vi "Retest_Continue_NO.vi"(8 "error in":errorcluster, 9 "Enable":bool=TRUE, 10 "input string":string, 11 "Text.Text Colors:BG Color":u32(colorbox)=16448250) -> (0 "error out":errorcluster, 1 "Boolean":bool, 2 "Continue 2":bool)   [LabVIEW 2021]
panel:
  in  "Continue":bool caption="Enter to continue"
  in  "Cancel":bool caption="ESC to No"
  in  "OK Button":bool caption="F3 to Retest"
  out "String":string
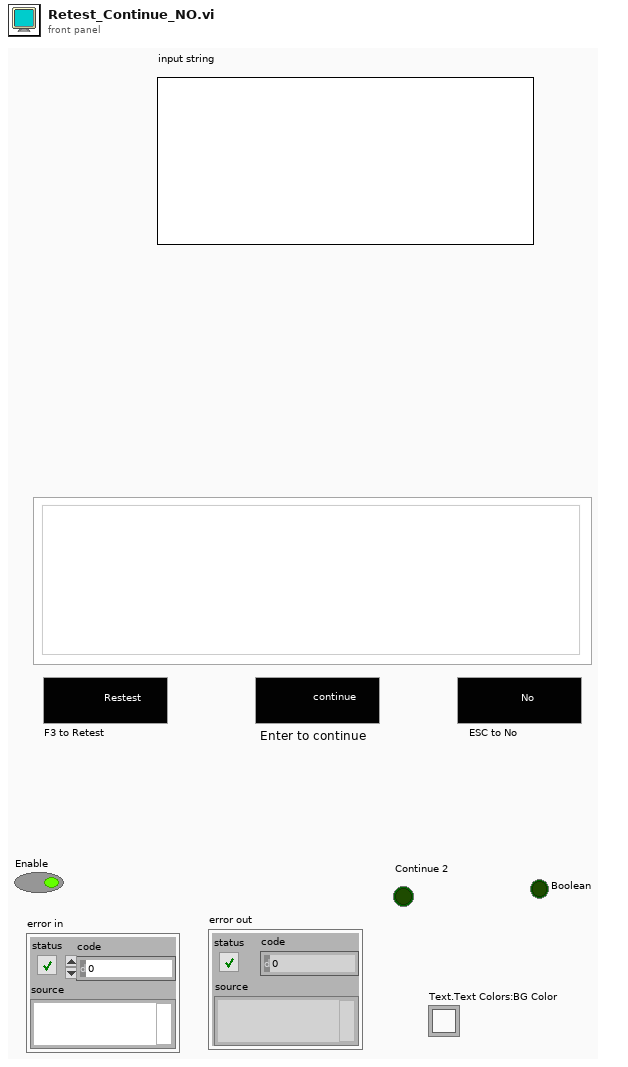
[diagram p1: front panel]
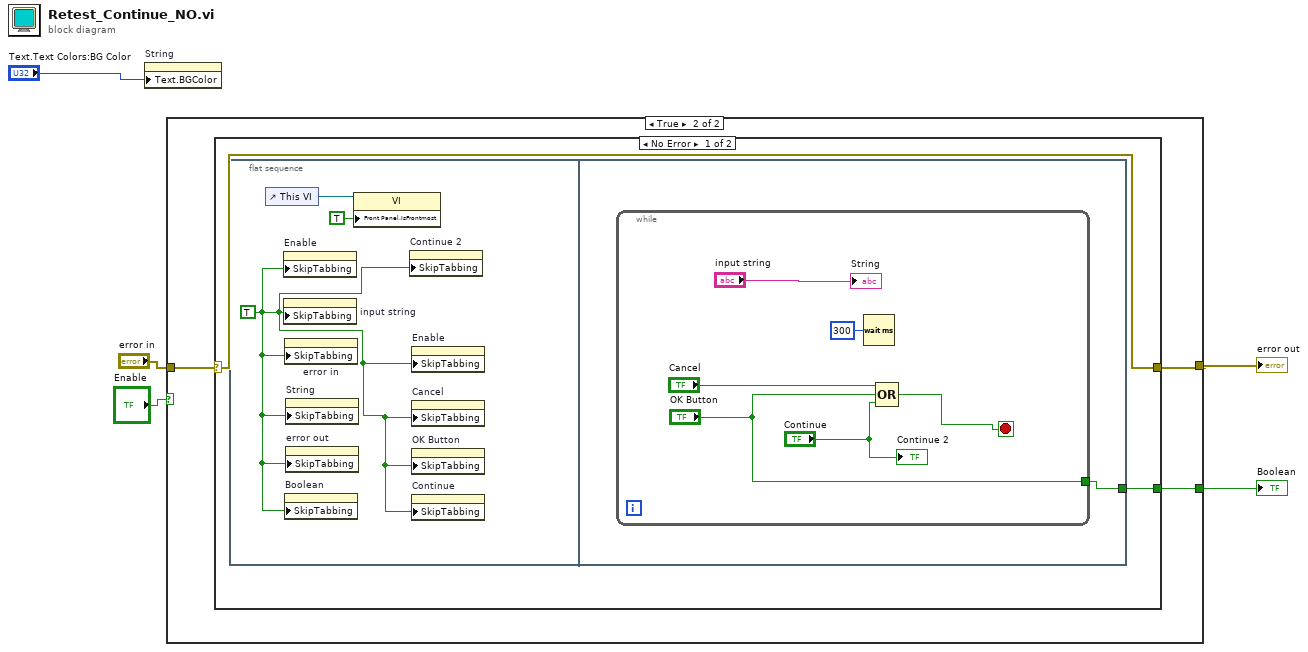
[diagram p0: block diagram]
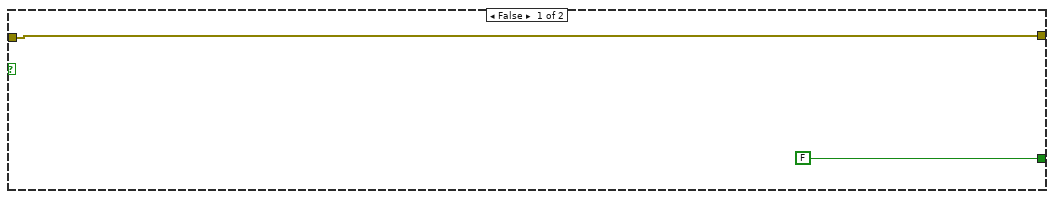
[diagram p2: hidden frame]
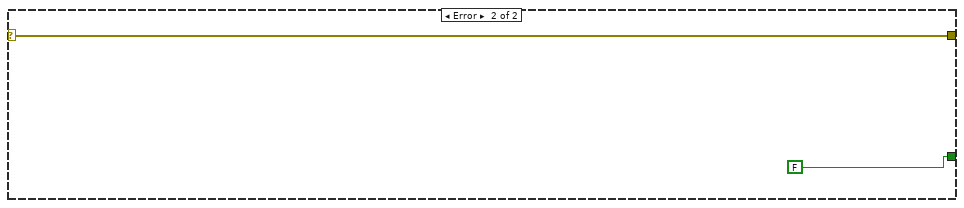
[diagram p3: hidden frame]
diagram:
  n1 = property on="String" class="Str"("Text.BGColor"="Text.Text Colors:BG Color") -> ()  [unwired: 2 in, 2 out]
  n2 = case shown="True" "Enable" {
    tunnel: "error in" -> [w7 w10]
    tunnel: [w7 w9] -> w4
    tunnel: [FALSE ("OK Button") w8] -> w2
    frame False {
    }
    frame True {
      n3 = case shown="No Error" w10 {
        selector: w10 -> [w12 w24]
        tunnel: [w12 w24] -> w9
        tunnel: [w11 FALSE ("OK Button")] -> w8
        frame No Error {
          n4 = flat-sequence {
            tunnel: [w16] -> w11
            frame #0 {
              w13 = TRUE ("Skip When Tabbing")
              n5 = control-ref of="This VI"() -> (w15:refnum<vi>)
              n6 = property on="Enable" class="Bool (strict)"("SkipTabbing"=w13) -> ()  [unwired: 2 in, 2 out]
              n7 = property on="input string" class="Str"("SkipTabbing"=w13) -> ()  [unwired: 2 in, 2 out]
              n8 = property on="error in" class="Clust (strict)"("SkipTabbing"=w13) -> ()  [unwired: 2 in, 2 out]
              n9 = property on="Boolean" class="Bool (strict)"("SkipTabbing"=w13) -> ()  [unwired: 2 in, 2 out]
              n10 = property on="String" class="Str"("SkipTabbing"=w13) -> ()  [unwired: 2 in, 2 out]
              n11 = property on="error out" class="Clust (strict)"("SkipTabbing"=w13) -> ()  [unwired: 2 in, 2 out]
              n12 = property class="VI"(reference=w15, "Front Panel.IsFrontmost"=TRUE ("Front Panel Window:Is Frontmost")) -> ()  [unwired: 1 in, 2 out]
              n13 = property on="Continue 2" class="Bool"("SkipTabbing"=w13) -> ()  [unwired: 2 in, 2 out]
              n14 = property on="Enable" class="Bool (strict)"("SkipTabbing"=w13) -> ()  [unwired: 2 in, 2 out]
              n15 = property on="Cancel" class="Bool"("SkipTabbing"=w13) -> ()  [unwired: 2 in, 2 out]
              n16 = property on="OK Button" class="Bool"("SkipTabbing"=w13) -> ()  [unwired: 2 in, 2 out]
              n17 = property on="Continue" class="Bool"("SkipTabbing"=w13) -> ()  [unwired: 2 in, 2 out]
            }
            frame #1 {
              n18 = while {
                tunnel: ["OK Button"] -> w16
                stop <- w18 stop-if-true
                n19 = Wait (ms)(milliseconds to wait=u32 300) -> ()  [unwired: 1 out]
                n20 = Compound Arithmetic op=OR("Cancel", "OK Button", "Continue") -> (w18:bool)
                "String" <- "input string"
                "Continue 2" <- "Continue"
              }
            }
          }
        }
        frame Error {
        }
      }
    }
  }
  "error out" <- w4
  "Boolean" <- w2
